vi "Prefix Array.vi"(6 "End Symbol":string, 7 "Start Symbol":string, 8 "error in (no error)":errorcluster, 10 "Array":string[](array[string]), 11 "JSON Serializer in":refnum<class "JSON Serializer.lvclass">) -> (0 "error out":errorcluster, 2 "String":string, 3 "JSON Serializer out":refnum<class "JSON Serializer.lvclass">)   [LabVIEW 2020, in "JKI JSON Serialization.lvlib" / "JSON Serializer.lvclass"]
uses:
  JSON Serializer.lvclass
  JSON Serializer.lvclass/JSON Serializer.ctl
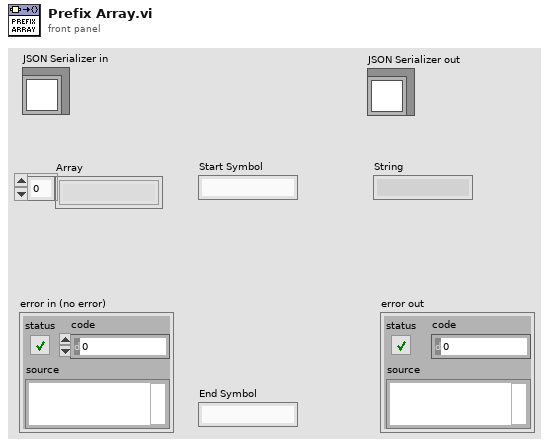
[diagram p1: front panel]
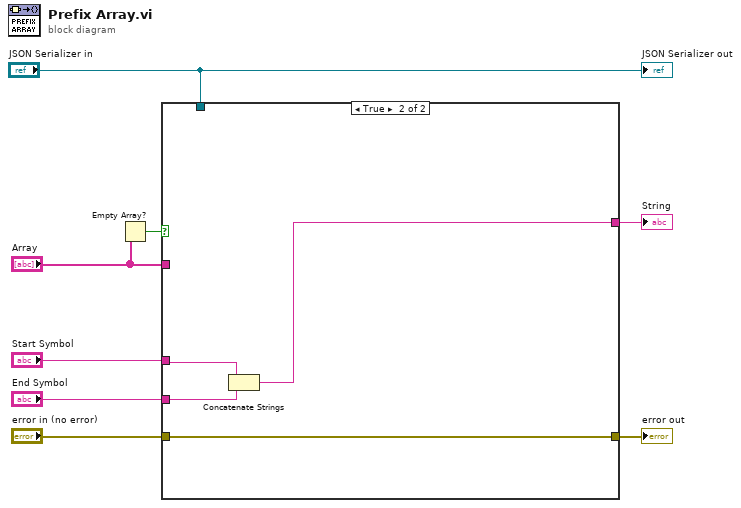
[diagram p0: block diagram]
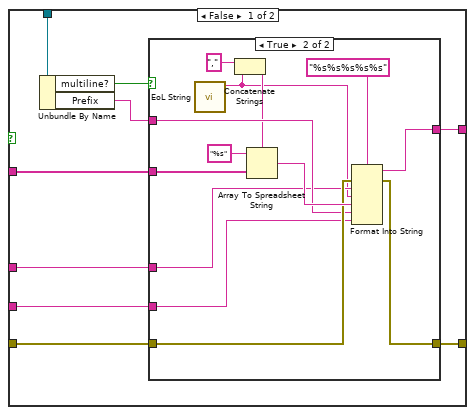
[diagram p2: hidden frame]
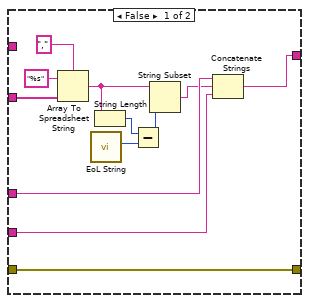
[diagram p3: hidden frame]
diagram:
  n1 = Empty Array?(array="Array") -> (empty?=w1:bool)
  n2 = case shown="True" w1 {
    tunnel: "error in (no error)" -> [w17 w43]
    tunnel: [w16 w43] -> w7
    tunnel: [w15 w44] -> w6
    tunnel: "Start Symbol" -> [w14 w46]
    tunnel: "End Symbol" -> [w13 w45]
    tunnel: "JSON Serializer in" -> [w12 _]
    tunnel: "Array" -> [w9 _]
    frame False {
      n3 = Unbundle By Name(w12) -> ("multiline?"=w11:bool, "Prefix"=w10:string)
      n4 = case shown="True" w11 {
        tunnel: w17 -> [w23 w41]
        tunnel: [w23 w40] -> w16
        tunnel: [w24 w39] -> w15
        tunnel: w9 -> [w27 w37]
        tunnel: w10 -> [_ w35]
        tunnel: w14 -> [w26 w31]
        tunnel: w13 -> [w25 w34]
        frame False {
          n5 = Array To Spreadsheet String(delimiter (Tab)=",", array=w27, 3:"%s" ("format string")) -> (spreadsheet string=w22:string)
          n6 = call "EoL String.vi"() -> ("EoL String Length"=w20:i32)  [unwired: 10 in, 1 out]
          n7 = String Length(string=w22) -> (length=w19:i32)
          n8 = Subtract(x=w19, y=w20) -> (x-y=w18:i32)
          n9 = String Subset(string=w22, length (rest)=w18) -> (substring=w21:string)  [unwired: 1 in]
          n10 = Concatenate Strings(w26, w21, w25) -> (w24:string)
        }
        frame True {
          n11 = call "EoL String.vi"() -> ("EoL String"=w30:string)  [unwired: 10 in, 1 out]
          n12 = Concatenate Strings("," ("delimiter (Tab)"), w30) -> (w32:string)
          n13 = Array To Spreadsheet String(delimiter (Tab)=w32, array=w37, 3:"%s" ("format string")) -> (spreadsheet string=w42:string)
          n14 = Format Into String(format string="%s%s%s%s%s", error in=w41, w31, w30, w42, w35, w34) -> (resulting string=w39:string, error out=w40:errorcluster)  [unwired: 1 in]
        }
      }
    }
    frame True {
      n15 = Concatenate Strings(w46, w45) -> (w44:string)
    }
  }
  "error out" <- w7
  "String" <- w6
  "JSON Serializer out" <- "JSON Serializer in"
